vi "Create Message Data Clusters (complex).vi"(8 "error in (no error)":errorcluster, 9 "generate serialization helpers":bool, 10 "message metadata":T1, 11 "library in":refnum<vi>) -> (0 "error out":errorcluster, 3 "library out":refnum<vi>)   [LabVIEW 2019, in "gRPC Template Creation Utility.lvlib"]
uses:
  gRPC Template Creation Utility.lvlib
  TypeDefs/Message Metadata (Scripting).ctl
  TypeDefs/Message Element Type.ctl
  TypeDefs/Message Element Metadata (Scripting).ctl
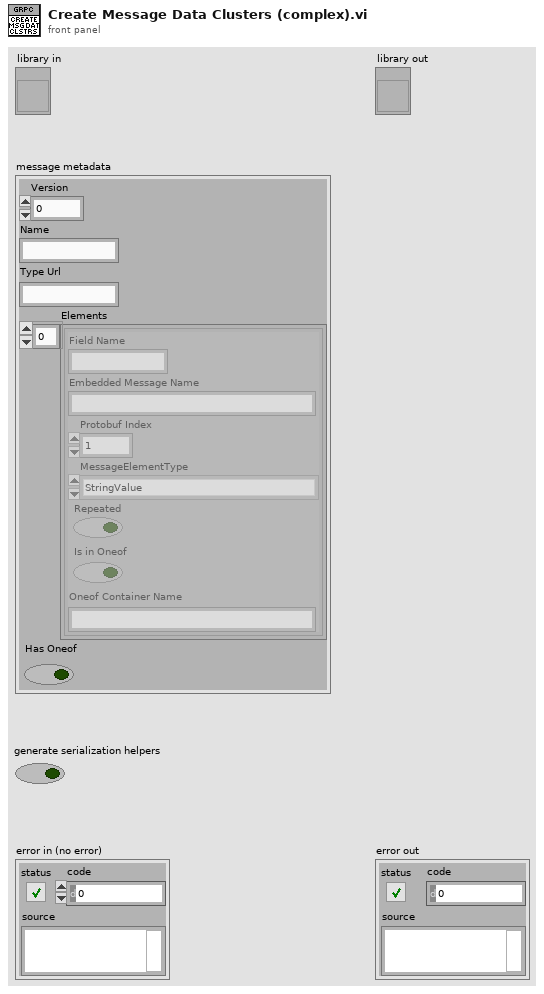
[diagram p1: front panel]
types:
  T1 = typedef "gRPC Template Creation Utility.lvlib/Message Metadata (Scripting).ctl" = cluster{"Version":i32, "Name":string, "Type Url":string, "Elements":T2[], "Has Oneof":bool}
  T2 = typedef "gRPC Template Creation Utility.lvlib/Message Element Metadata (Scripting).ctl" = cluster{"Field Name":string, "Embedded Message Name":string, "Protobuf Index":i32, "MessageElementType":T3, "Repeated":bool, "Is in Oneof":bool, "Oneof Container Name":string}
  T3 = typedef "gRPC Template Creation Utility.lvlib/Message Element Type.ctl" = enum32{"Int32Value", "FloatValue", "DoubleValue", "BoolValue", "StringValue", "MessageValue", "Int64Value", "UInt32Value", "UInt64Value", "EnumValue", "Bytes", "Fixed64", "Fixed32", "SFixed64", "SFixed32", "SInt64", "SInt32"}
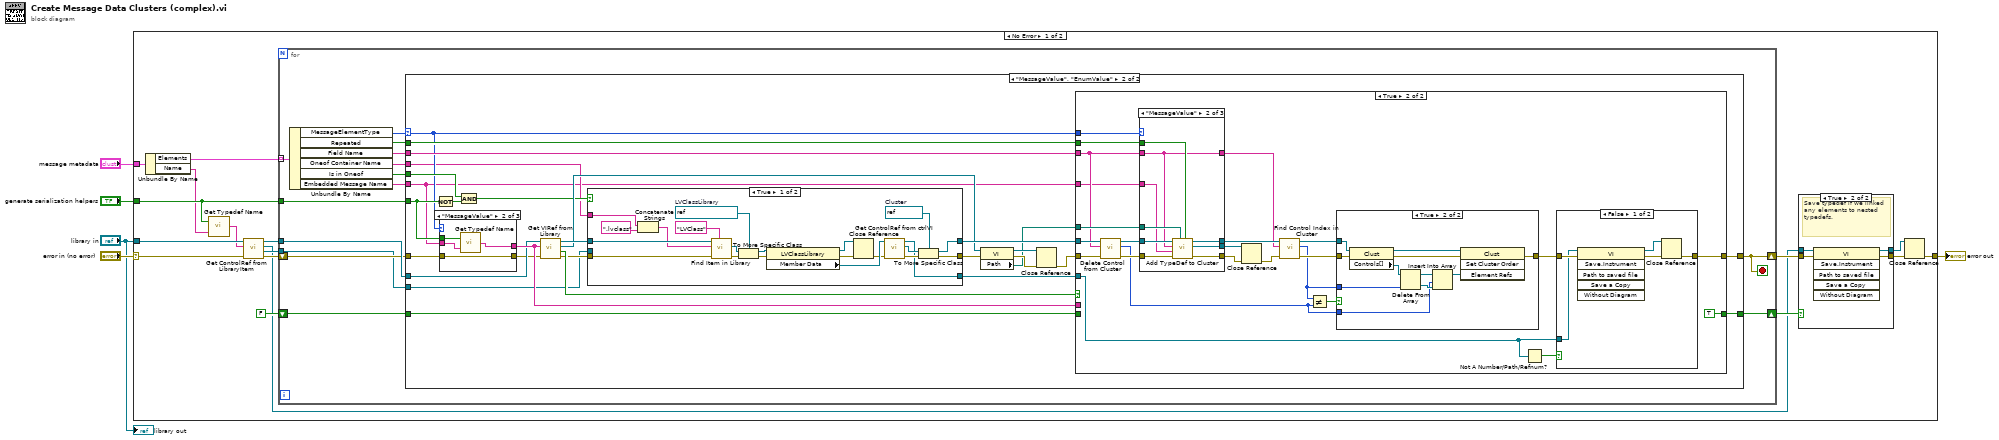
[diagram p0: block diagram]
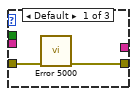
[diagram p4: hidden frame]
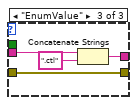
[diagram p5: hidden frame]
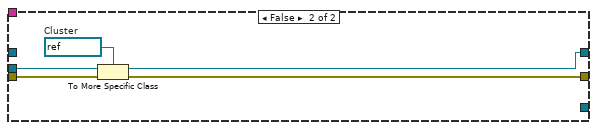
[diagram p6: hidden frame]
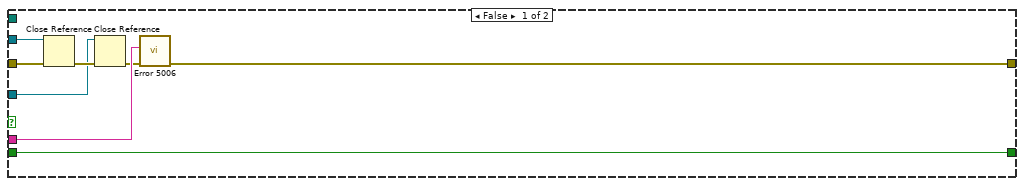
[diagram p7: hidden frame]
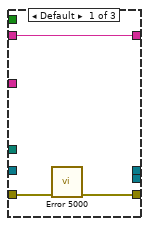
[diagram p9: hidden frame]
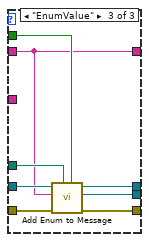
[diagram p10: hidden frame]
diagram:
  n1 = case shown="No Error" "error in (no error)" {
    selector: "error in (no error)" -> [w18 w179]
    tunnel: "message metadata" -> [w22 _]
    tunnel: "library in" -> [w16 _]
    tunnel: [w8 w179] -> w4
    tunnel: "generate serialization helpers" -> [w20 _]
    frame No Error {
      n2 = Unbundle By Name(w22) -> ("Elements"=w21:T2[], "Name"=w19:string)
      n3 = call "Get Typedef Name.vi"("embedded message name"=w19, "generate serialization helpers"=w20) -> ("typedef name"=w14:string)
      n4 = call "Get ControlRef from LibraryItem.vi"("error in (no error)"=w18, "Control Name"=w14, "Library item in"=w16) -> ("error out"=w17:errorcluster, "Control ref out"=w13:refnum<vi>, "VI ref out"=w6:refnum<vi>, "Library item out"=w15:refnum<vi>)  [unwired: 4 in, 1 out]
      n5 = for {
        tunnel: w21 -> [w41] mode=indexing
        shift-right: [w39] -> w10
        shift-left: w17 -> [w40]
        tunnel: w20 -> [w38]
        tunnel: w15 -> [w42]
        tunnel: w13 -> [w31]
        shift-right: [w29] -> w11
        shift-left: FALSE ("generate serialization helpers") -> [w30]
        stop <- w39 stop-if-true
        n6 = Unbundle By Name(w41) -> ("MessageElementType"=w34:T3, "Repeated"=w37:bool, "Field Name"=w36:string, "Oneof Container Name"=w35:string, "Is in Oneof"=w32:bool, "Embedded Message Name"=w33:string)
        n7 = case shown="\"MessageValue\", \"EnumValue\"" w34 {
          selector: w34 -> [_ w53]
          tunnel: w42 -> [_ w50]
          tunnel: w40 -> [w44 w54]
          tunnel: [w44 w60] -> w39
          tunnel: w38 -> [_ w67]
          tunnel: w37 -> [_ w57]
          tunnel: w36 -> [_ w56]
          tunnel: w32 -> [_ w55]
          tunnel: w35 -> [_ w52]
          tunnel: w33 -> [_ w51]
          tunnel: w31 -> [_ w48]
          tunnel: w30 -> [w43 w47]
          tunnel: [w43 w46] -> w29
          frame Default {
          }
          frame "MessageValue", "EnumValue" {
            n8 = Not(x=w67) -> (.not. x?=w66:bool)
            n9 = case shown="\"MessageValue\"" w53 {
              tunnel: [_ w78 w80] -> w72
              tunnel: w67 -> [_ w77 _]
              tunnel: w51 -> [_ w76 w81]
              tunnel: w54 -> [w74 w75 w79]
              tunnel: [w73 w75 w79] -> w49
              frame Default {
                n10 = call "Error 5000.vi"("error in (no error)"=w74) -> ("error out"=w73:errorcluster)  [unwired: 10 in]
              }
              frame "MessageValue" {
                n11 = call "Get Typedef Name.vi"("embedded message name"=w76, "generate serialization helpers"=w77) -> ("typedef name"=w78:string)
              }
              frame "EnumValue" {
                n12 = Concatenate Strings(w81, ".ctl" ("string")) -> (w80:string)
              }
            }
            n13 = And(x=w55, y=w66) -> (x .and. y?=w58:bool)
            n14 = call "Get VIRef from Library.vi"("error in (no error)"=w49, "item name"=w72, "library in"=w50) -> ("error out"=w69:errorcluster, "found"=w70:bool, "vi"=w65:refnum<vi>, "library out"=w68:refnum<vi>)  [unwired: 5 in]
            n15 = case shown="True" w58 {
              tunnel: w48 -> [_ w108]
              tunnel: [w94 w106] -> w71
              tunnel: w69 -> [w101 w105]
              tunnel: [w88 w104] -> w61
              tunnel: w68 -> [w103 _]
              tunnel: w52 -> [w93 _]
              tunnel: [w83 _] -> w45
              frame True {
                w95 = refnum<vi> refnum  # Cluster
                w100 = refnum<vi> refnum  # LVClassLibrary
                n16 = Concatenate Strings(w93, ".lvclass" ("string")) -> (w91:string)
                n17 = call "Find Item in Library.vi"("Item Type"="LVClass", "error in (no error)"=w101, "Item Name"=w91, "Library item in"=w103) -> ("error out"=w99:errorcluster, "Project Item (Library Item)"=w98:refnum<vi>)  [unwired: 4 in, 2 out]
                n18 = To More Specific Class(target class=w100, reference=w98, error in=w99) -> (specific class reference=w97:refnum<vi>, error out=w96:errorcluster)
                n19 = property class="LVClassLibrary"(reference=w97, error in=w96) -> (reference out=w86:refnum<vi>, error out=w85:errorcluster, "Member Data"=w90:refnum<vi>)
                n20 = Close Reference(reference=w86, error in (no error)=w85) -> (error out=w84:errorcluster)
                n21 = call "Get ControlRef from ctrlVI.vi"("error in (no error)"=w84, "VI ref in"=w90) -> ("error out"=w87:errorcluster, "Control ref out"=w89:refnum<vi>, "VI ref out"=w83:refnum<vi>)  [unwired: 7 in]
                n22 = To More Specific Class(target class=w95, reference=w89, error in=w87) -> (specific class reference=w94:refnum<vi>, error out=w88:errorcluster)
              }
              frame False {
                w107 = refnum<vi> refnum  # Cluster
                n23 = To More Specific Class(target class=w107, reference=w108, error in=w105) -> (specific class reference=w106:refnum<vi>, error out=w104:errorcluster)
              }
            }
            n24 = property class="VI"(reference=w65, error in=w61) -> (reference out=w63:refnum<vi>, error out=w64:errorcluster, "Path"=w59:path)
            n25 = Close Reference(reference=w63, error in (no error)=w64) -> (error out=w62:errorcluster)
            n26 = case shown="True" w70 {
              tunnel: w71 -> [w116 w140]
              tunnel: [w114 w118] -> w60
              tunnel: w62 -> [w115 w135]
              tunnel: w56 -> [_ w124]
              tunnel: w57 -> [_ w127]
              tunnel: w72 -> [w113 _]
              tunnel: w59 -> [_ w126]
              tunnel: w53 -> [_ w125]
              tunnel: w51 -> [_ w122]
              tunnel: w47 -> [w112 _]
              tunnel: [w112 TRUE ("generate serialization helpers")] -> w46
              tunnel: w45 -> [w109 w117]
              frame False {
                n27 = Close Reference(reference=w116, error in (no error)=w115) -> (error out=w111:errorcluster)
                n28 = Close Reference(reference=w109, error in (no error)=w111) -> (error out=w110:errorcluster)
                n29 = call "Error 5006.vi"("error in (no error)"=w110, "Embedded Message Name"=w113) -> ("error out"=w114:errorcluster)  [unwired: 9 in]
              }
              frame True {
                n30 = call "Delete Control from Cluster.vi"("error in (no error)"=w135, "Control Name in"=w124, "Cluster ref in"=w140) -> ("error out"=w134:errorcluster, "Deleted Index"=w128:i32, "Cluster ref out"=w133:refnum<vi>)  [unwired: 6 in]
                n31 = case shown="\"MessageValue\"" w125 {
                  tunnel: w134 -> [w149 w158 w166]
                  tunnel: w133 -> [_ w157 w162]
                  tunnel: [_ w156 w164] -> w132
                  tunnel: [_ w155 w163] -> w131
                  tunnel: [w148 w154 w165] -> w130
                  tunnel: w127 -> [_ w153 w161]
                  tunnel: w126 -> [_ w152 w160]
                  tunnel: w124 -> [w147 w151 w159]
                  tunnel: [w147 w151 w159] -> w123
                  tunnel: w122 -> [_ w150 _]
                  frame Default {
                    n32 = call "Error 5000.vi"("error in (no error)"=w149) -> ("error out"=w148:errorcluster)  [unwired: 10 in]
                  }
                  frame "MessageValue" {
                    n33 = call "Add TypeDef to Cluster.vi"("isArray (F)"=w153, "TypeDef path"=w152, "error in (no error)"=w158, "field message name"=w150, "Field Name"=w151, "Owning cluster ref in"=w157) -> ("error out"=w154:errorcluster, "Control ref out"=w155:refnum<vi>, "Owning cluster ref out"=w156:refnum<vi>)  [unwired: 3 in]
                  }
                  frame "EnumValue" {
                    n34 = call "Add Enum to Message.vi"("isArray (F)"=w161, "TypeDef path"=w160, "error in (no error)"=w166, "Field Name"=w159, "Owning cluster ref in"=w162) -> ("error out"=w165:errorcluster, "Control ref out"=w163:refnum<vi>, "Owning cluster ref out"=w164:refnum<vi>)  [unwired: 4 in]
                  }
                }
                n35 = Close Reference(reference=w131, error in (no error)=w130) -> (error out=w129:errorcluster)
                n36 = call "Find Control Index in Cluster.vi"("error in (no error)"=w129, "Control Name"=w123, "Cluster ref in"=w132) -> ("error out"=w137:errorcluster, "Control Index"=w136:i32, "Cluster ref out"=w138:refnum<vi>)  [unwired: 6 in]
                n37 = Not Equal?(x=w136, y=w128) -> (x != y?=w139:bool)
                n38 = case shown="True" w139 {
                  tunnel: w138 -> [_ w178]
                  tunnel: w137 -> [w167 w177]
                  tunnel: w136 -> [_ w176]
                  tunnel: w128 -> [_ w173]
                  tunnel: [w167 w168] -> w120
                  frame False {
                  }
                  frame True {
                    n39 = property class="Clust"(reference=w178, error in=w177) -> (reference out=w172:refnum<vi>, error out=w169:errorcluster, "Controls[]"=w170:refnum<vi>[])
                    n40 = Delete From Array(array=w170, index=w176) -> (deleted portion=w174:refnum<vi>, array with subset deleted=w175:refnum<vi>[])  [unwired: 1 in]
                    n41 = Insert Into Array(array=w175, index=w173, new element=w174) -> (w171:refnum<vi>[])
                    n42 = invoke class="Clust" method="Set Cluster Order"(reference=w172, error in=w169, "Element Refs"=w171) -> (error out=w168:errorcluster)  [unwired: 1 in, 3 out]
                  }
                }
                n43 = Not A Number/Path/Refnum?(number/path/refnum=w117) -> (NaN/Path/Refnum?=w119:bool)
                n44 = case shown="False" w119 {
                  tunnel: w120 -> [w145 w146]
                  tunnel: [w141 w146] -> w118
                  tunnel: w117 -> [w144 _]
                  frame False {
                    n45 = invoke class="VI" method="Save.Instrument"(reference=w144, error in=w145) -> (reference out=w142:refnum<vi>, error out=w143:errorcluster)  [unwired: 4 in, 4 out]
                    n46 = Close Reference(reference=w142, error in (no error)=w143) -> (error out=w141:errorcluster)
                  }
                  frame True {
                  }
                }
              }
            }
          }
        }
      }
      n47 = case shown="True" w11 {
        tunnel: w10 -> [w24 w28]
        tunnel: [w24 w27] -> w9
        tunnel: [w23 w26] -> w7
        tunnel: w6 -> [w23 w25]
        frame False {
        }
        frame True {
          # "Save typedef if we linked any elements to nested typedefs."
          n48 = invoke class="VI" method="Save.Instrument"(reference=w25, error in=w28) -> (reference out=w26:refnum<vi>, error out=w27:errorcluster)  [unwired: 4 in, 4 out]
        }
      }
      n49 = Close Reference(reference=w7, error in (no error)=w9) -> (error out=w8:errorcluster)
    }
    frame Error {
    }
  }
  "error out" <- w4
  "library out" <- "library in"
